vi "Ajout_event.vi"(1 "Type de segment":u8, 2 "Evennements_entrée":T1, 3 "Température":dbl[](array[numeric]), 4 "Instant":dbl[](array[numeric])) -> (0 "Evennements_sortie":T1)   [LabVIEW 2022 SP3]
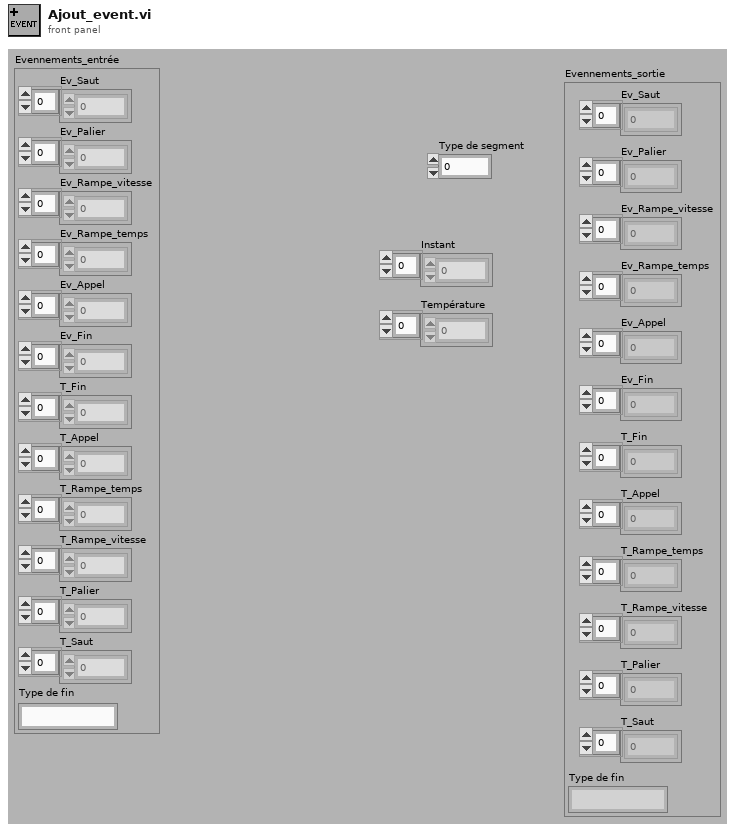
[diagram p1: front panel]
types:
  T1 = cluster{"Ev_Saut":dbl[], "Ev_Palier":dbl[], "Ev_Rampe_vitesse":dbl[], "Ev_Rampe_temps":dbl[], "Ev_Appel":dbl[], "Ev_Fin":dbl[], "T_Fin":dbl[], "T_Appel":dbl[], "T_Rampe_temps":dbl[], "T_Rampe_vitesse":dbl[], "T_Palier":dbl[], "T_Saut":dbl[], "Type de fin":string}
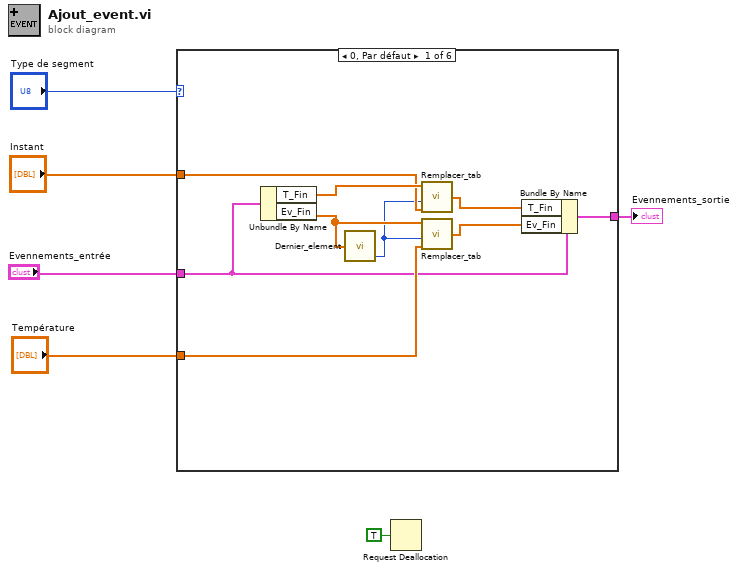
[diagram p0: block diagram]
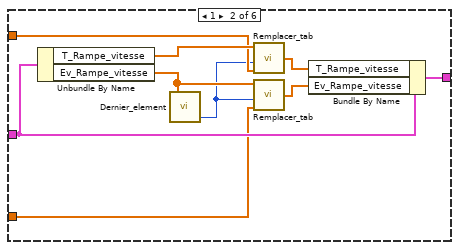
[diagram p2: hidden frame]
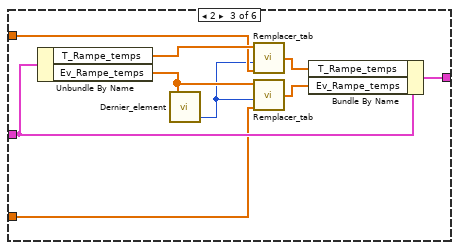
[diagram p3: hidden frame]
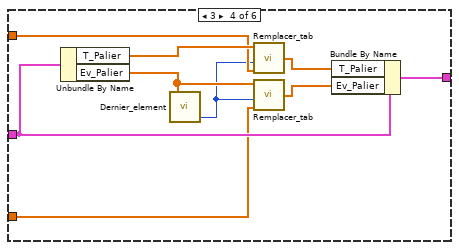
[diagram p4: hidden frame]
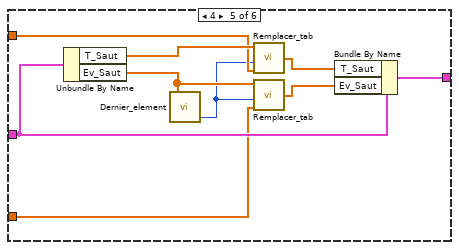
[diagram p5: hidden frame]
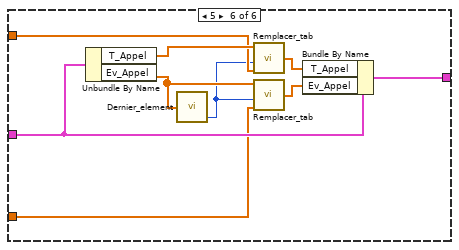
[diagram p6: hidden frame]
diagram:
  n1 = case shown="0, Par défaut" "Type de segment" {
    tunnel: "Evennements_entrée" -> [w7 w20 w29 w38 w47 w56]
    tunnel: [w11 w19 w28 w37 w46 w55] -> w2
    tunnel: "Instant" -> [w10 w18 w27 w36 w45 w54]
    tunnel: "Température" -> [w9 w17 w26 w35 w44 w53]
    frame 0, Default {
      n2 = Unbundle By Name(w7) -> ("T_Fin"=w14:dbl[], "Ev_Fin"=w15:dbl[])
      n3 = call "Dernier_element.vi"("Tableau en entrée"=w15) -> ("Taille/Indice N+1"=w8:i32)  [unwired: 2 out]
      n4 = call "Remplacer_tab.vi"("Nouvel élément/sous tableau"=w10, "A partir de"=w8, "Tableau"=w14) -> ("Tableau inséré/remplacé"=w12:dbl[])  [unwired: 1 in]
      n5 = call "Remplacer_tab.vi"("Nouvel élément/sous tableau"=w9, "A partir de"=w8, "Tableau"=w15) -> ("Tableau inséré/remplacé"=w13:dbl[])  [unwired: 1 in]
      n6 = Bundle By Name(cluster=w7, "T_Fin"=w12, "Ev_Fin"=w13) -> (w11:T1)
    }
    frame 1 {
      n7 = Unbundle By Name(w20) -> ("T_Rampe_vitesse"=w23:dbl[], "Ev_Rampe_vitesse"=w24:dbl[])
      n8 = call "Dernier_element.vi"("Tableau en entrée"=w24) -> ("Taille/Indice N+1"=w16:i32)  [unwired: 2 out]
      n9 = call "Remplacer_tab.vi"("Nouvel élément/sous tableau"=w18, "A partir de"=w16, "Tableau"=w23) -> ("Tableau inséré/remplacé"=w21:dbl[])  [unwired: 1 in]
      n10 = call "Remplacer_tab.vi"("Nouvel élément/sous tableau"=w17, "A partir de"=w16, "Tableau"=w24) -> ("Tableau inséré/remplacé"=w22:dbl[])  [unwired: 1 in]
      n11 = Bundle By Name(cluster=w20, "T_Rampe_vitesse"=w21, "Ev_Rampe_vitesse"=w22) -> (w19:T1)
    }
    frame 2 {
      n12 = Unbundle By Name(w29) -> ("T_Rampe_temps"=w32:dbl[], "Ev_Rampe_temps"=w33:dbl[])
      n13 = call "Dernier_element.vi"("Tableau en entrée"=w33) -> ("Taille/Indice N+1"=w25:i32)  [unwired: 2 out]
      n14 = call "Remplacer_tab.vi"("Nouvel élément/sous tableau"=w27, "A partir de"=w25, "Tableau"=w32) -> ("Tableau inséré/remplacé"=w30:dbl[])  [unwired: 1 in]
      n15 = call "Remplacer_tab.vi"("Nouvel élément/sous tableau"=w26, "A partir de"=w25, "Tableau"=w33) -> ("Tableau inséré/remplacé"=w31:dbl[])  [unwired: 1 in]
      n16 = Bundle By Name(cluster=w29, "T_Rampe_temps"=w30, "Ev_Rampe_temps"=w31) -> (w28:T1)
    }
    frame 3 {
      n17 = Unbundle By Name(w38) -> ("T_Palier"=w41:dbl[], "Ev_Palier"=w42:dbl[])
      n18 = call "Dernier_element.vi"("Tableau en entrée"=w42) -> ("Taille/Indice N+1"=w34:i32)  [unwired: 2 out]
      n19 = call "Remplacer_tab.vi"("Nouvel élément/sous tableau"=w36, "A partir de"=w34, "Tableau"=w41) -> ("Tableau inséré/remplacé"=w39:dbl[])  [unwired: 1 in]
      n20 = call "Remplacer_tab.vi"("Nouvel élément/sous tableau"=w35, "A partir de"=w34, "Tableau"=w42) -> ("Tableau inséré/remplacé"=w40:dbl[])  [unwired: 1 in]
      n21 = Bundle By Name(cluster=w38, "T_Palier"=w39, "Ev_Palier"=w40) -> (w37:T1)
    }
    frame 4 {
      n22 = Unbundle By Name(w47) -> ("T_Saut"=w50:dbl[], "Ev_Saut"=w51:dbl[])
      n23 = call "Dernier_element.vi"("Tableau en entrée"=w51) -> ("Taille/Indice N+1"=w43:i32)  [unwired: 2 out]
      n24 = call "Remplacer_tab.vi"("Nouvel élément/sous tableau"=w45, "A partir de"=w43, "Tableau"=w50) -> ("Tableau inséré/remplacé"=w48:dbl[])  [unwired: 1 in]
      n25 = call "Remplacer_tab.vi"("Nouvel élément/sous tableau"=w44, "A partir de"=w43, "Tableau"=w51) -> ("Tableau inséré/remplacé"=w49:dbl[])  [unwired: 1 in]
      n26 = Bundle By Name(cluster=w47, "T_Saut"=w48, "Ev_Saut"=w49) -> (w46:T1)
    }
    frame 5 {
      n27 = Unbundle By Name(w56) -> ("T_Appel"=w59:dbl[], "Ev_Appel"=w60:dbl[])
      n28 = call "Dernier_element.vi"("Tableau en entrée"=w60) -> ("Taille/Indice N+1"=w52:i32)  [unwired: 2 out]
      n29 = call "Remplacer_tab.vi"("Nouvel élément/sous tableau"=w54, "A partir de"=w52, "Tableau"=w59) -> ("Tableau inséré/remplacé"=w57:dbl[])  [unwired: 1 in]
      n30 = call "Remplacer_tab.vi"("Nouvel élément/sous tableau"=w53, "A partir de"=w52, "Tableau"=w60) -> ("Tableau inséré/remplacé"=w58:dbl[])  [unwired: 1 in]
      n31 = Bundle By Name(cluster=w56, "T_Appel"=w57, "Ev_Appel"=w58) -> (w55:T1)
    }
  }
  "Evennements_sortie" <- w2
  n32 = Request Deallocation(TRUE ("flag")) -> ()
